vi "JY .vi"() -> ()   [LabVIEW 2018]
doc: "This VI is an example on how to use the HORIBA Jobin Yvon Monochromator control VIs. To use this VI, press the Run button in LabVIEW.\n\nThe VI will retreive all configured monochromators from the computer's resgistry.\n\nSelect the desired monochromator from the Mono ID combo box and press the Connect button to start communications with that device. If the Force Initialization button is enabled, the monochromator will start its automatic calibration routine. If the Force Initialization button is not enabled, the sofwtare will keep the monochromator in its current positions.\n\nAfter connecting to the instrumnet, the VI will retreive the current positions of all movable motors in the system. This will continue until the Move To Target Position or Stop buttons are pressed.\n\nMove to Target Positions will move the monochromator to the postions entered in the indicators of the VI.\n\nStop will stop running the VI."
uses:
  <vilib>/Utility/file.llb/Write Delimited Spreadsheet (DBL).vi
panel:
  out "最终存储路径":path
  in  "Commande tab":enum32{"Settings", "Trigger In", "Infos"}(tab)
  in  "Integration time (ms) :":i16=10
  in  "Number of Areas :":u16=1 min=1 step=1
  in  "ADC":u16(ring) caption="Device Name" items=["20 kHz       ", " 1 MHz       ", " 1 MHz Ultra "]
  in  "GAIN":u16(ring) caption="Device Name" items=["High Light", "Best Dynamic Range", "High Sensitivity"]
  in  "Device Name":u16(ring) items=["Synapse CCD (Lateral)", "Synapse_IGA (Axial)"]
  out "Uniques ID":u16(ring) items=["CCD1", "CCD2"]
  in  "Reformat":bool
  in  "Signal type :":enum16{"TTL Rising Edge", "TTL Falling Edge"}(ring)=enum."TTL Falling Edge"
  in  "Trigger Type :":enum16{"On Start", "Per Acquisition"}(ring)
  in  "Enable InputTriggers :":bool
  out "DataSize":i32=262144
  out "Y Pixels:":i32=256
  out "X Pixels:":i32=1024
  out "Firmware\nVersion":string="V1.20 CCD_4000"
  out "Intensity Graph":dbl[][](graph)
  out "initialized ccd":bool
  in  "Continuous":bool
  in  "CCD Busy":bool
  out "indicator":string
  in  "Close":bool=TRUE
  in  "Setup":bool
  in  "Temperature":bool
  in  "Acquire":bool
  in  "Shutter Enable":bool=TRUE
  out "Acq Time(ms)":u32=2010
  in  "initialize":bool
  in  "Target\nFront Entrance":dbl
  in  "Exit Mirror":u16(ring)=3 caption="Target Position Exit Mirror" items=["Front"=2, "Side"=3]
  in  "Entrance Mirror":u16(ring)=2 caption="Target Position\nEntrance Mirror" items=["Front"=2, "Side"=3]
  in  "Target Grating":string(combo)="2"
  in  "Target WL":dbl=898.0
  in  "Move To\nTarget Positions":bool
  out "Units":string="nm"
  in  "Connect":bool
  out "Initialized JY":bool=TRUE
  out "Current UniqueID":string="Mono4"
  in  "Force\nInitialization":bool=TRUE
  out "Units":string="mm"
  out "Front Entrance":dbl
  out "Exit Mirror\nPosition":i32(ring)=2 items=["EntranceMirror", "ExitMirror", "Front", "Side"]
  out "Entrance Mirror\nPosition":i32(ring)=2 items=["EntranceMirror", "ExitMirror", "Front", "Side"]
  out "Current Description":string="1" caption="Description"
  out "Grating Index":i32=1
  out "Current Grating":dbl=1200.0
  out "Current WL":dbl=897.9988
  in  "Mono ID":string(combo)="Mono1"
  in  "trigEventString":string
  in  "trigSigTypeString":string
  in  "trigAddress":i32
  out "ADC Number":i32[](array[numeric])=[0, 1, 2, 3, 4]
  out "Gain Number":i32[](array[numeric])=[10, 11, 12, 13, 8, 2]
  out "temp graph":dbl(graph)=66.11766439999997
  out "areas :":i32[][](array[numeric])=[[1], [1], [1], [1024], [256], [1], [1]]
  out "Gratings":dbl[](array[numeric])=[1200.0, 300.0]
  out "error out":errorcluster
  # "JY Control"
  # "Setup"
  # "Grating / Wavelength Control"
  # "Slits"
  # "Swing Mirrors"
  # "CCD Control"
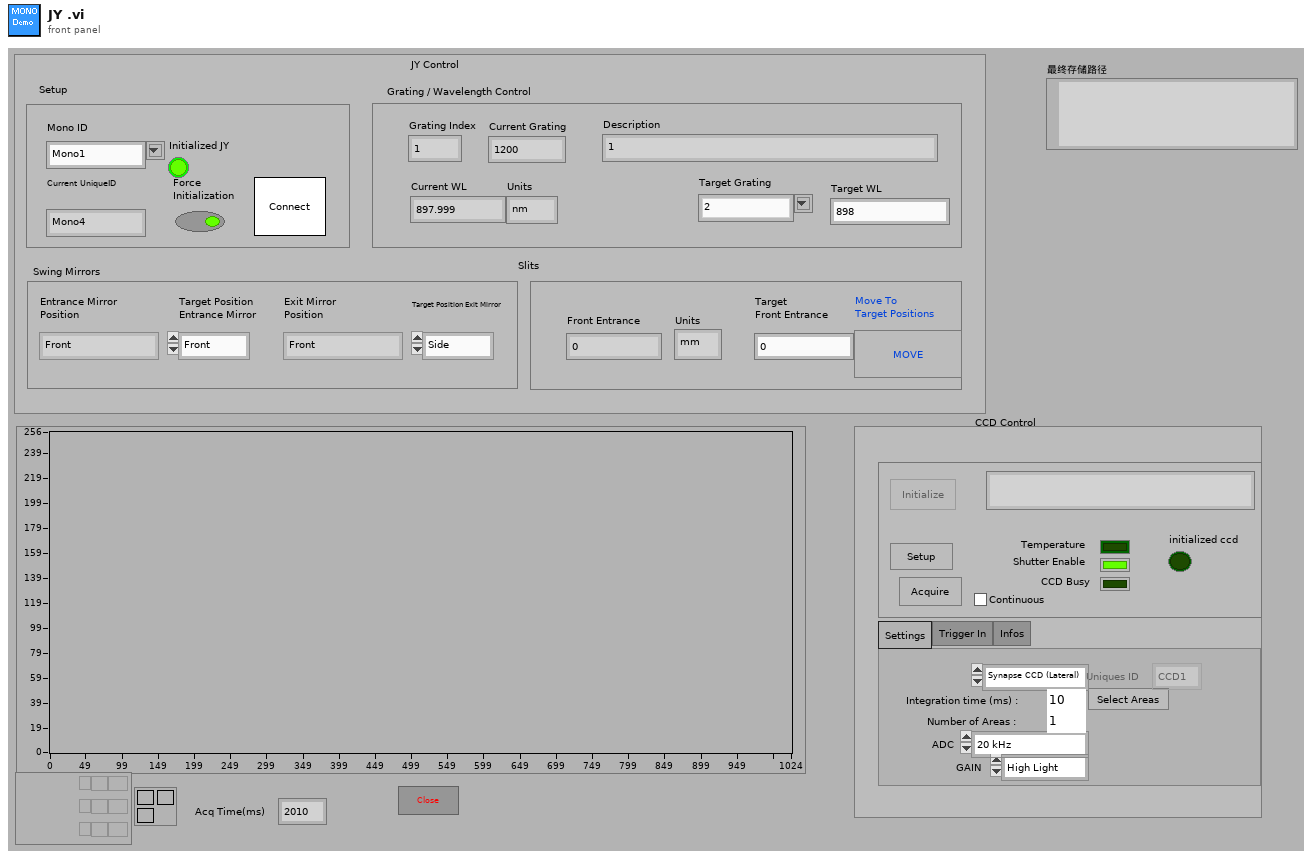
[diagram p1: front panel]
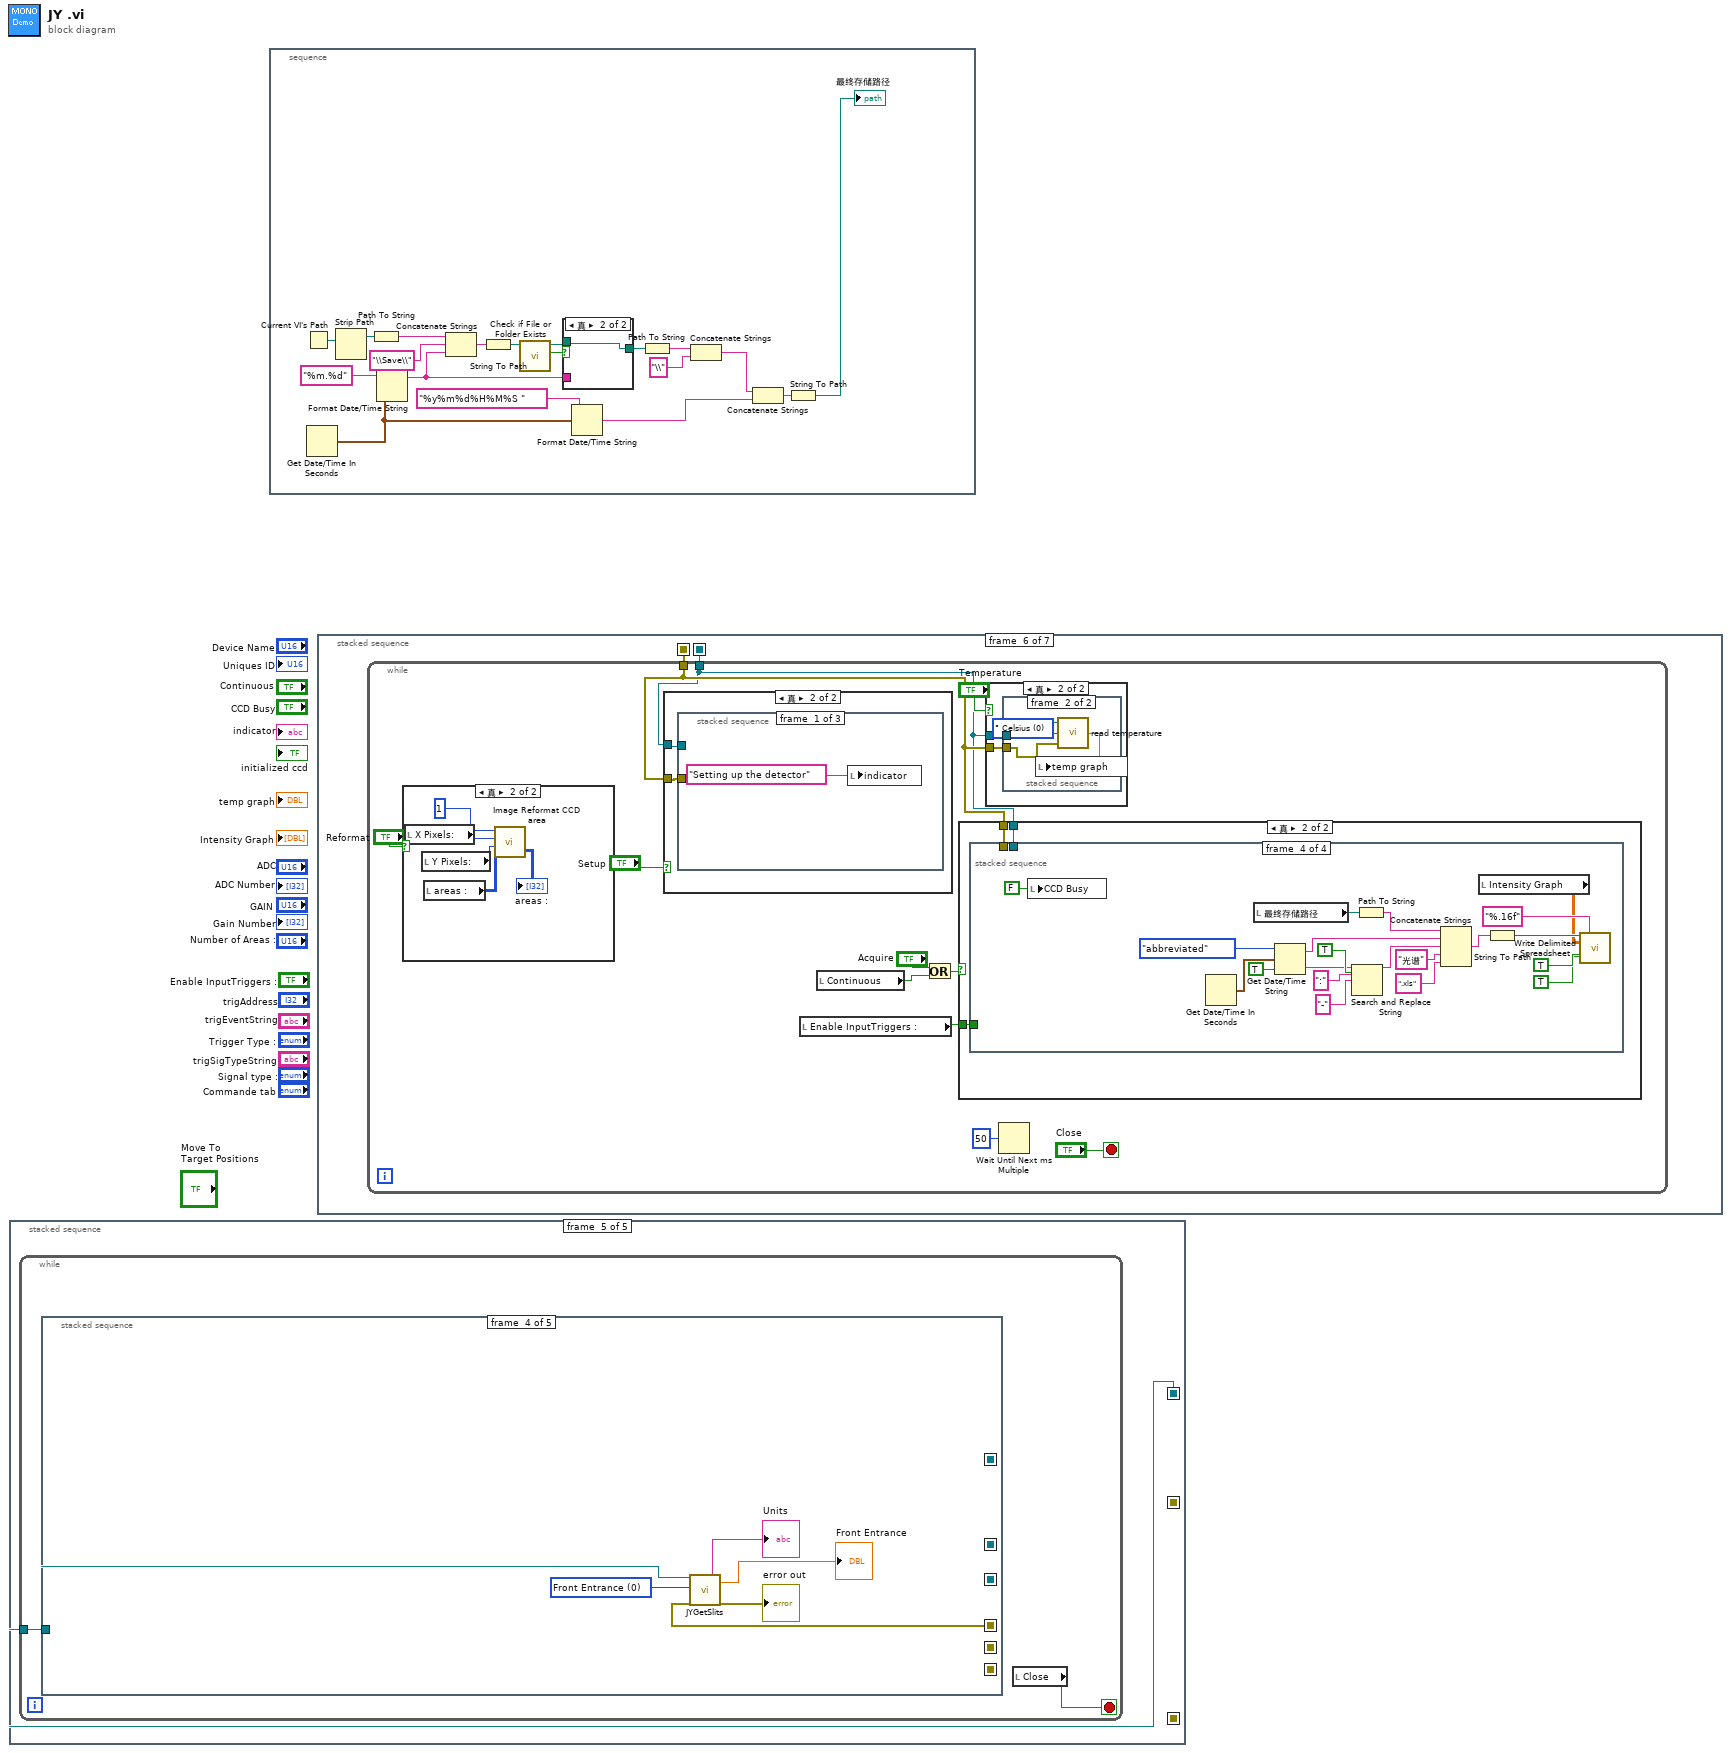
[diagram p0: block diagram]
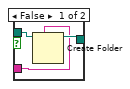
[diagram p2: hidden frame]
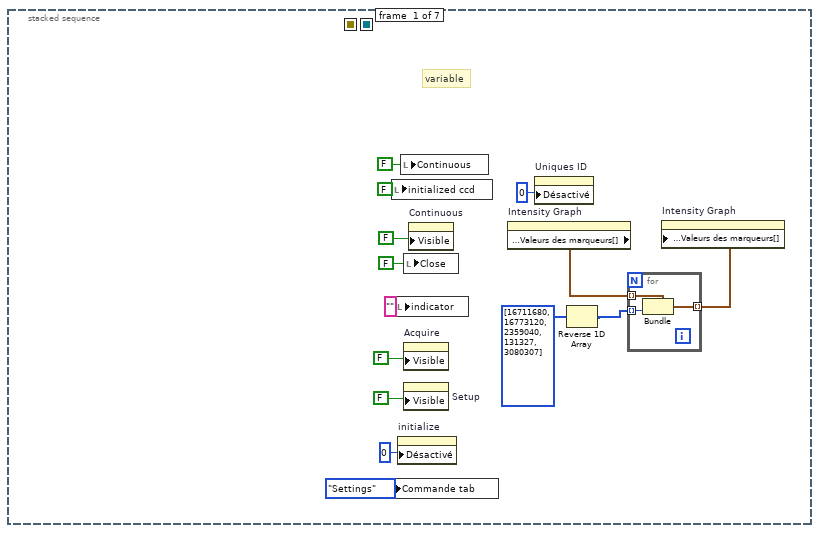
[diagram p3: hidden frame]
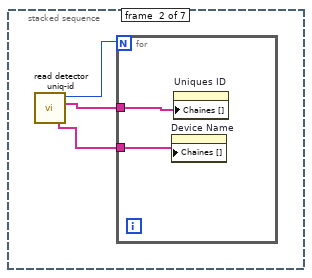
[diagram p4: hidden frame]
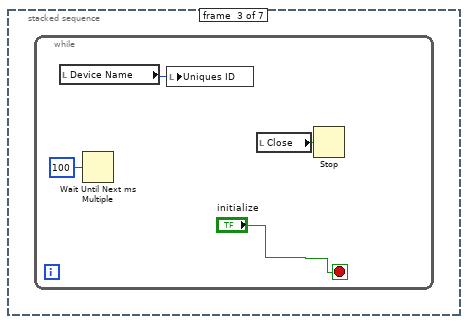
[diagram p5: hidden frame]
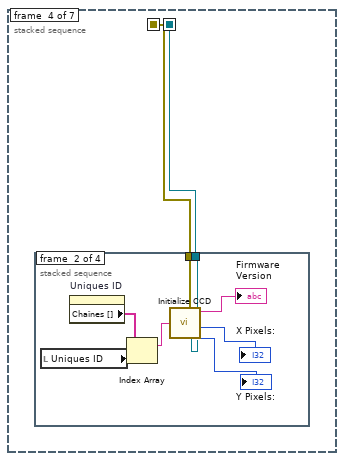
[diagram p6: hidden frame]
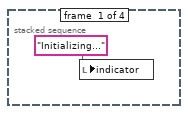
[diagram p7: hidden frame]
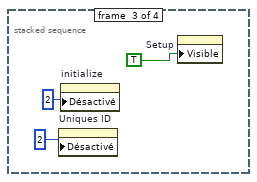
[diagram p8: hidden frame]
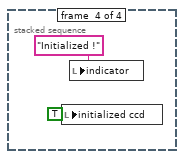
[diagram p9: hidden frame]
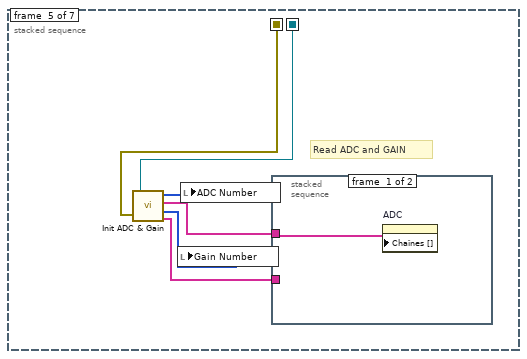
[diagram p10: hidden frame]
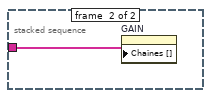
[diagram p11: hidden frame]
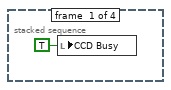
[diagram p13: hidden frame]
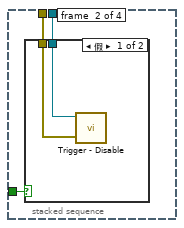
[diagram p14: hidden frame]
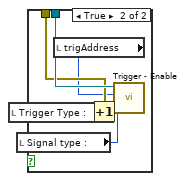
[diagram p15: hidden frame]
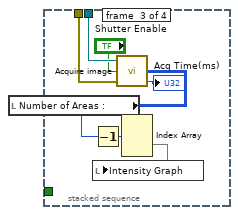
[diagram p16: hidden frame]
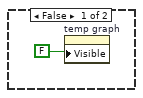
[diagram p17: hidden frame]
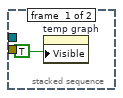
[diagram p18: hidden frame]
diagram:
  n1 = stacked-sequence {
    seq-local: [_ _ w10 _ _] -> [_ _ _ w20 w25]
    seq-local: [_ _ w9 _ _] -> [_ _ _ w19 _]
    seq-local: [_ _ _ w18 _] -> [_ _ _ _ _]
    frame #0 {
      n2 = call "Get Monos From Config Browser.vi"() -> ("UniqueIDs"=w5:string[], "Mono ID"=w6:string[])  [unwired: 3 in, 1 out]
      n3 = Build Cluster Array(w6, w5) -> (w3:cluster{"String":string, "String":string}[])
      n4 = property on="Mono ID" class="CmbBox"("Strings And Values []"=w3) -> ()  [unwired: 2 in, 2 out]
      n5 = Index Array(array=w3, index=0) -> (element=w4:cluster{"String":string, "String":string})
      n6 = Unbundle(w4) -> ("String"=w1:string)  [unwired: 1 out]
      "Current UniqueID" <- w1
      n7 = local write "Mono ID"(w1) -> ()
    }
    frame #1 {
      n8 = while {
        stop <- "Connect" stop-if-true
        n9 = local read "Mono ID"() -> (w7:string)
        n10 = local write "Current UniqueID"(w7) -> ()
      }
    }
    frame #2 {
      n11 = local read "Mono ID"() -> (w12:string)
      n12 = call "JYInitMono.vi"("Unique ID"=w12, "Force Init"="Force\nInitialization") -> ("Refnum out"=w10:refnum<k7>, "Initialized"=→"Initialized JY":bool, "error out"=w9:errorcluster)  [unwired: 9 in, 2 out]
    }
    frame #3 {
      n13 = call "Show Current Grating.vi"("Refnum in"=w20, "error in (no error)"=w19) -> ("Gratings"=w21:dbl[], "Grating Index"=w15:i32, "Current Grating"=w17:dbl, "Current Description"=w14:string, "error out"=w18:errorcluster)  [unwired: 5 in, 4 out]
      "Gratings" <- w21
      n14 = local write "Current Grating"(w17) -> ()
      n15 = local write "Current Description"(w14) -> ()
      n16 = Number To Decimal String(number=w21) -> (decimal integer string=w23:string[])  [unwired: 1 in]
      n17 = Number To Decimal String(number=w15) -> (decimal integer string=w16:string)  [unwired: 1 in]
      n18 = property on="Target Grating" class="CmbBox"("Value"=w16) -> ()  [unwired: 2 in, 2 out]
      n19 = Build Cluster Array(w23, string[] ["1", "2", "3"]) -> (w24:cluster{"Numeric":string, string}[])
      n20 = property on="Target Grating" class="CmbBox"("Strings And Values []"=w24) -> ()  [unwired: 2 in, 2 out]
    }
    frame #4 {
      n21 = while {
        tunnel: w25 -> [w27]
        stop <- w26 stop-if-true
        n22 = stacked-sequence {
          seq-local: [w31 _ _ _ _] -> [_ w38 w49 _ w56]
          seq-local: [w30 _ _ _ _] -> [_ w37 w48 _ _]
          seq-local: [_ w36 _ _ _] -> [_ _ _ _ _]
          seq-local: [_ w35 _ _ _] -> [_ _ _ _ _]
          seq-local: [_ _ w41 _ _] -> [_ _ _ _ _]
          seq-local: [_ _ w40 _ _] -> [_ _ _ w51 _]
          tunnel: w27 -> [w29 _ _ w52 _]
          frame #0 {
            n23 = call "Show Current Grating.vi"("Refnum in"=w29) -> ("Grating Index"=→"Grating Index":i32, "Current Grating"=→"Current Grating":dbl, "Current Description"=→"Current Description":string, "error out"=w30:errorcluster, "JYMONOLib.IJYMonoReqd"=w31:refnum<k7>)  [unwired: 6 in, 4 out]
          }
          frame #1 {
            n24 = call "JYGetCurrentWL.vi"("error in (no error)"=w37, "JYMONOLib.IJYMonoReqd"=w38) -> ("error out"=w35:errorcluster, "Units"=→"Units":string, "Current WL"=→"Current WL":dbl, "JYMONOLib.IJYMonoReqd 2"=w36:refnum<k7>)  [unwired: 6 in]
          }
          frame #2 {
            w46 = u16 1 items=["Entrance", "Exit"] ("Mirror Number")
            w47 = u16 0 items=["Entrance", "Exit"] ("Mirror Number")
            n25 = call "JYGetMirrorPos.vi"("error in (no error)"=w48, "Mirror"=w47, "Refnum In"=w49) -> ("error out"=w44:errorcluster, "Current Mirror Position"=→"Entrance Mirror\nPosition":i32, "Refnum Out"=w45:refnum<k7>)  [unwired: 1 in]
            n26 = call "JYGetMirrorPos.vi"("error in (no error)"=w44, "Mirror"=w46, "Refnum In"=w45) -> ("error out"=w40:errorcluster, "Current Mirror Position"=→"Exit Mirror\nPosition":i32, "Refnum Out"=w41:refnum<k7>)  [unwired: 1 in]
          }
          frame #3 {
            w54 = u16 0 items=["Front Entrance", "Side Entrance", "Front Exit", "Side Exit", "First Intermediate", "Second Intermediate"] ("Slit")
            n27 = call "JYGetSlits.vi"("MonoRefNum IN"=w52, "Slit"=w54, "error in (no error)"=w51) -> ("Units"=→"Units":string, "Slit Width"=→"Front Entrance":dbl, "error out"=→"error out":errorcluster)  [unwired: 13 in, 1 out]
          }
          frame #4 {
            n28 = local read "Move To\nTarget Positions"() -> (w57:bool)
            n29 = case shown="真" w57 {
              tunnel: w56 -> [_ w58]
              frame False {
              }
              frame True {
                n30 = stacked-sequence {
                  seq-local: [w60 _ _ _] -> [_ w66 _ _]
                  seq-local: [_ w64 _ _] -> [_ _ w81 _]
                  seq-local: [_ _ w68 _] -> [_ _ _ w87]
                  seq-local: [_ _ _ w84] -> [_ _ _ _]
                  tunnel: w58 -> [w62 w65 w79 w88]
                  frame #0 {
                    n31 = property on="Target Grating" class="CmbBox"() -> ("Value"=w59:string)  [unwired: 2 in, 2 out]
                    n32 = local read "error out"() -> (w61:errorcluster)
                    n33 = Decimal String To Number(string=w59) -> (number=w63:i32)  [unwired: 2 in, 1 out]
                    n34 = call "JYTurret.vi"("error in (no error)"=w61, "Grating Index"=w63, "JYMONOLib.IJYMonoReqd"=w62) -> ("error out"=w60:errorcluster)  [unwired: 2 out]
                  }
                  frame #1 {
                    # "Move Grating to Target Position"
                    n35 = call "JYMoveToWavelength.vi"("error in (no error)"=w66, "Target WL"="Target WL", "RefNum In"=w65) -> ("error out"=w64:errorcluster)  [unwired: 1 in, 2 out]
                  }
                  frame #2 {
                    w74 = u16 1 items=["Entrance", "Exit"] ("Mirror Number")
                    w73 = u16 0 items=["Entrance", "Exit"] ("Mirror Number")
                    w80 = u16 1 items=["Entrance", "Exit", "Front", "Side"] ("Mirror Number")
                    w83 = u16 0 items=["Entrance", "Exit", "Front", "Side"] ("Mirror Number")
                    # "Move Mirrors"
                    n36 = call "JYMirrorMove.vi"("error in (no error)"=w81, "Mirror Position"="Entrance Mirror", "Mirror Number"=w83, "RefNum In"=w79) -> ("error out"=w78:errorcluster)  [unwired: 6 in, 1 out]
                    n37 = call "JYMirrorMove.vi"("error in (no error)"=w78, "Mirror Position"="Exit Mirror", "Mirror Number"=w80, "RefNum In"=w79) -> ("error out"=w71:errorcluster, "MonoRefNum Out"=w72:refnum<k7>)  [unwired: 6 in]
                    n38 = call "JYGetMirrorPos.vi"("error in (no error)"=w71, "Mirror"=w73, "Refnum In"=w72) -> ("error out"=w76:errorcluster, "Current Mirror Position"=w70:i32, "Refnum Out"=w75:refnum<k7>)  [unwired: 1 in]
                    n39 = local write "Entrance Mirror\nPosition"(w70) -> ()
                    n40 = call "JYGetMirrorPos.vi"("error in (no error)"=w76, "Mirror"=w74, "Refnum In"=w75) -> ("error out"=w68:errorcluster, "Current Mirror Position"=w69:i32)  [unwired: 1 in, 1 out]
                    n41 = local write "Exit Mirror\nPosition"(w69) -> ()
                  }
                  frame #3 {
                    w86 = u16 0 items=["Front Entrance", "Side Entrance", "Front Exit", "Side Exit", "First Intermediate", "Second Intermediate"] ("Slit")
                    # "Set New Slit Positions"
                    n42 = call "JYSlits.vi"("JYMONOLib.IJYMonoReqd"=w88, "Slit"=w86, "error in (no error)"=w87, "Slit Width"="Target\nFront Entrance") -> ("error out"=w84:errorcluster)  [unwired: 1 in, 1 out]
                  }
                }
              }
            }
          }
        }
        n43 = local read "Close"() -> (w26:bool)
      }
    }
  }
  n44 = stacked-sequence {
    frame #0 {
      n45 = Current VI's Path() -> (path=w105:path)
      n46 = Get Date/Time In Seconds() -> (seconds since 1Jan1904=w102:timestamp)
      n47 = Strip Path(path=w105) -> (stripped path=w104:path)  [unwired: 1 out]
      n48 = Path To String(path=w104) -> (string=w101:string)
      n49 = Format Date/Time String(time format string (%c)="%m.%d" ("时间格式字符串(%c)"), seconds (now)=w102) -> (date/time string=w94:string)  [unwired: 1 in]
      n50 = Concatenate Strings(w101, "\\Save\\" ("字符串"), w94) -> (w99:string)
      n51 = String To Path(string=w99) -> (path=w98:path)
      n52 = call <vilib>:"Check if File or Folder Exists.vi"("path"=w98) -> ("file or folder exists?"=w97:bool, "dup path"=w95:path)  [unwired: 8 in, 1 out]
      n53 = case shown="真" w97 {
        tunnel: [w110 w111] -> w96
        tunnel: w95 -> [w109 w111]
        tunnel: w94 -> [w108 _]
        frame False {
          n54 = Create Folder(prompt (Create Folder)=w108, path (use dialog)=w109) -> (created path=w110:path)  [unwired: 1 in, 2 out]
        }
        frame True {
        }
      }
      n55 = Format Date/Time String(time format string (%c)="%y%m%d%H%M%S " ("时间格式字符串(%c)"), seconds (now)=w102) -> (date/time string=w90:string)  [unwired: 1 in]
      n56 = Path To String(path=w96) -> (string=w93:string)
      n57 = Concatenate Strings(w93, "\\" ("字符串")) -> (w91:string)
      n58 = Concatenate Strings(w91, w90) -> (w107:string)
      n59 = String To Path(string=w107) -> (path=→"最终存储路径":path)
    }
  }
  n60 = stacked-sequence {
    seq-local: [_ _ _ w139 _ _ _] -> [_ _ _ _ w155 w163 w249]
    seq-local: [_ _ _ w138 _ _ _] -> [_ _ _ _ w154 w162 w250]
    frame #0 {
      # "variable"
      n61 = local write "Commande tab"(enum32{"Settings", "Trigger In", "Infos"}."Settings" ("Commande tab")) -> ()
      n62 = local write "initialized ccd"(FALSE ("initialized ?")) -> ()
      n63 = local write "indicator"("" ("indicator")) -> ()
      n64 = property on="initialize" class="Bool"("Désactivé"=u8 0) -> ()  [unwired: 2 in, 2 out]
      n65 = local write "Continuous"(FALSE ("Continuous")) -> ()
      n66 = local write "Close"(FALSE ("Close")) -> ()
      n67 = property on="Acquire" class="Bool"("Visible"=FALSE) -> ()  [unwired: 2 in, 2 out]
      n68 = property on="Setup" class="Bool"("Visible"=FALSE) -> ()  [unwired: 2 in, 2 out]
      n69 = property on="Continuous" class="Bool (严格)"("Visible"=FALSE) -> ()  [unwired: 2 in, 2 out]
      n70 = property on="Intensity Graph" class="IntGraph (严格)"() -> ("Échelle des Z.Valeurs des marqueurs[]"=w115:cluster{dbl, u32}[])  [unwired: 2 in, 2 out]
      n71 = property on="Uniques ID" class="Ring (严格)"("Désactivé"=u8 0) -> ()  [unwired: 2 in, 2 out]
      n72 = Reverse 1D Array(array=u32[] [16711680, 16773120, 2359040, 131327, 3080307] ("Sous-tableau")) -> (reversed array=w116:u32[])
      n73 = for {
        tunnel: w116 -> [w128] mode=indexing
        tunnel: [w127] -> w114 mode=indexing
        tunnel: w115 -> [w126] mode=indexing
        n74 = Bundle(cluster=w126, w128) -> (w127:cluster{dbl, u32})  [unwired: 1 out]
      }
      n75 = property on="Intensity Graph" class="IntGraph (严格)"("Échelle des Z.Valeurs des marqueurs[]"=w114) -> ()  [unwired: 2 in, 2 out]
    }
    frame #1 {
      n76 = call <userlib>:"read detector uniq-id.vi"() -> ("nbr of components"=w131:i32, "UniqueID"=w130:string[], "Name"=w129:string[])  [unwired: 4 out]
      n77 = for {
        N: w131 -> [_]
        tunnel: w130 -> [w133]
        tunnel: w129 -> [w132]
        n78 = property on="Device Name" class="Ring (严格)"("Chaînes []"=w132) -> ()  [unwired: 2 in, 2 out]
        n79 = property on="Uniques ID" class="Ring (严格)"("Chaînes []"=w133) -> ()  [unwired: 2 in, 2 out]
      }
    }
    frame #2 {
      n80 = while {
        stop <- "initialize" stop-if-true
        n81 = local read "Device Name"() -> (w136:u16)
        n82 = Wait Until Next ms Multiple(millisecond multiple=u32 100 ("n millisecondes")) -> ()  [unwired: 1 out]
        n83 = local write "Uniques ID"(w136) -> ()
        n84 = local read "Close"() -> (w134:bool)
        n85 = Stop(stop? (T)=w134) -> ()
      }
    }
    frame #3 {
      n86 = stacked-sequence {
        tunnel: [_ w145 _ _] -> w139
        tunnel: [_ w144 _ _] -> w138
        frame #0 {
          n87 = local write "indicator"("Initializing..." ("indicator")) -> ()
        }
        frame #1 {
          n88 = local read "Uniques ID"() -> (w142:u16)
          n89 = property on="Uniques ID" class="Ring (严格)"() -> ("Chaînes []"=w143:string[])  [unwired: 2 in, 2 out]
          n90 = Index Array(array=w143, index=w142) -> (element=w141:string)
          n91 = call <userlib>:"Initialize CCD.vi"("Unique id:"=w141) -> ("activeYPixels"=→"Y Pixels:":i32, "JYCCDLib.IJYCCDReqd"=w144:refnum<k7>, "activeXPixels"=→"X Pixels:":i32, "sortie d'erreur"=w145:errorcluster, "FirmwareVersion"=→"Firmware\nVersion":string)  [unwired: 3 out]
        }
        frame #2 {
          n92 = property on="Uniques ID" class="Ring (严格)"("Désactivé"=u8 2) -> ()  [unwired: 2 in, 2 out]
          n93 = property on="initialize" class="Bool"("Désactivé"=u8 2) -> ()  [unwired: 2 in, 2 out]
          n94 = property on="Setup" class="Bool"("Visible"=TRUE) -> ()  [unwired: 2 in, 2 out]
        }
        frame #3 {
          n95 = local write "initialized ccd"(TRUE ("initialized ?")) -> ()
          n96 = local write "indicator"("Initialized !" ("indicator")) -> ()
        }
      }
    }
    frame #4 {
      # "Read ADC and GAIN"
      n97 = call <userlib>:"Init ADC & Gain.vi"("JYCCDLib.IJYCCDReqd"=w154, "input error"=w155) -> ("ADC Number"=w157:i32[], "ADC description"=w159:string[], "Gain Number"=w156:i32[], "Gain description"=w158:string[])
      n98 = local write "Gain Number"(w156) -> ()
      n99 = local write "ADC Number"(w157) -> ()
      n100 = stacked-sequence {
        tunnel: w159 -> [w160 _]
        tunnel: w158 -> [_ w161]
        frame #0 {
          n101 = property on="ADC" class="Ring (严格)"("Chaînes []"=w160) -> ()  [unwired: 2 in, 2 out]
        }
        frame #1 {
          n102 = property on="GAIN" class="Ring (严格)"("Chaînes []"=w161) -> ()  [unwired: 2 in, 2 out]
        }
      }
    }
    frame #5 {
      n103 = while {
        tunnel: w162 -> [w165]
        tunnel: w163 -> [w166]
        stop <- "Close" stop-if-true
        n104 = case shown="真" "Reformat" {
          frame False {
          }
          frame True {
            n105 = local read "X Pixels:"() -> (w228:i32)
            n106 = local read "Y Pixels:"() -> (w230:i32)
            n107 = local read "areas :"() -> (w226:i32[][])
            n108 = call "Image Reformat CCD area.vi"("areas :"=w226, "Y Pixels:"=w230, "X Pixels:"=w228, "numAreas"=1) -> ("areas"=→"areas :":i32[][])  [unwired: 1 out]
          }
        }
        n109 = case shown="真" "Setup" {
          tunnel: w166 -> [_ w231]
          tunnel: w165 -> [_ w232]
          frame False {
          }
          frame True {
            n110 = stacked-sequence {
              tunnel: w231 -> [_ w246 _]
              tunnel: w232 -> [_ w243 _]
              frame #0 {
                n111 = local write "indicator"("Setting up the detector" ("indicator")) -> ()
              }
              frame #1 {
                w244 = 1 items=["JYMCD_ACQ_FORMAT_IMAGE", "JYMCD_ACQ_FORMAT_SCAN"] ("Acquisition type")
                n112 = local read "Gain Number"() -> (w238:i32[])
                n113 = local read "GAIN"() -> (w234:u16)
                n114 = local read "ADC Number"() -> (w239:i32[])
                n115 = local read "ADC"() -> (w235:u16)
                n116 = Index Array(array=w238, index=w234) -> (element=w236:i32)
                n117 = Index Array(array=w239, index=w235) -> (element=w237:i32)
                n118 = local read "Number of Areas :"() -> (w241:u16)
                n119 = local read "areas :"() -> (w242:i32[][])
                n120 = call <userlib>:"Setup CCD.vi"("numAreas"=w241, "areas :"=w242, "JYCCDLib.IJYCCDReqd"=w243, "entrée d'erreur (pas d'erreur)"=w246, "Acquisition type"=w244, "Gain"=w236, "Select ADC"=w237, "Integration time(ms)"="Integration time (ms) :") -> ("DataSize"=→"DataSize":i32)  [unwired: 1 out]
              }
              frame #2 {
                w247 = TRUE ("Visible")
                n121 = property on="Acquire" class="Bool"("Visible"=w247) -> ()  [unwired: 2 in, 2 out]
                n122 = local write "indicator"("Ready !" ("indicator")) -> ()
                n123 = property on="Continuous" class="Bool (严格)"("Visible"=w247) -> ()  [unwired: 2 in, 2 out]
              }
            }
          }
        }
        n124 = local read "Enable InputTriggers :"() -> (w164:bool)
        n125 = local read "Continuous"() -> (w167:bool)
        n126 = Or(x="Acquire", y=w167) -> (x .or. y?=w169:bool)
        n127 = case shown="真" w169 {
          tunnel: w165 -> [_ w177]
          tunnel: w166 -> [_ w176]
          tunnel: w164 -> [_ w175]
          frame False {
          }
          frame True {
            n128 = stacked-sequence {
              tunnel: w177 -> [_ w180 w197 _]
              tunnel: w176 -> [_ w179 w196 _]
              tunnel: w175 -> [_ w181 _ _]
              frame #0 {
                n129 = local write "CCD Busy"(TRUE ("CCD Busy")) -> ()
              }
              frame #1 {
                n130 = case shown="假" w181 {
                  tunnel: w180 -> [w183 w189]
                  tunnel: w179 -> [w182 w188]
                  frame False {
                    n131 = call <userlib>:"Trigger - Disable.vi"("Error In"=w182, "JYCCDLib.IJYCCDReqd"=w183) -> ()  [unwired: 6 out]
                  }
                  frame True {
                    n132 = local read "Trigger Type :"() -> (w186:enum16{"On Start", "Per Acquisition"})
                    n133 = local read "Signal type :"() -> (w185:enum16{"TTL Rising Edge", "TTL Falling Edge"})
                    n134 = local read "trigAddress"() -> (w187:i32)
                    n135 = Increment(x=w186) -> (x+1=w184:enum16{"On Start", "Per Acquisition"})
                    n136 = call <userlib>:"Trigger - Enable.vi"("Error In"=w188, "sigType"=w185, "event"=w184, "trigAddress"=w187, "JYCCDLib.IJYCCDReqd"=w189) -> ()  [unwired: 3 out]
                  }
                }
              }
              frame #2 {
                n137 = local read "Number of Areas :"() -> (w191:u16)
                n138 = Decrement(x=w191) -> (x-1=w193:u16)
                n139 = call "Acquire image.vi"("error in"=w196, "ShutterOpen"="Shutter Enable", "JYCCDLib.IJYCCDReqd"=w197) -> ("Acq Time(ms)"=→"Acq Time(ms)":u32, "Datas"=w194:i32[][][])  [unwired: 1 out]
                n140 = Index Array(array=w194, index (dim 0)=w193) -> (element=w192:i32[][])  [unwired: 2 in]
                n141 = local write "Intensity Graph"(w192) -> ()
              }
              frame #3 {
                n142 = local write "CCD Busy"(FALSE ("CCD Busy")) -> ()
                n143 = Get Date/Time In Seconds() -> (seconds since 1Jan1904=w206:timestamp)
                n144 = local read "最终存储路径"() -> (w215:path)
                n145 = Get Date/Time String(date format (0)=enum16{"short", "long", "abbreviated"}."abbreviated" ("日期格式(0)"), seconds (now)=w206, want seconds? (F)=TRUE ("需要秒？(F)")) -> (date string=w214:string, time string=w209:string)
                n146 = Search and Replace String(replace all?=TRUE ("替换全部？(F)"), input string=w209, search string=":" ("搜索字符串"), replace string="-" ("替换字符串(\"\")")) -> (result string=w213:string)  [unwired: 4 in, 3 out]
                n147 = Path To String(path=w215) -> (string=w216:string)
                n148 = Concatenate Strings(w216, w214, w213, "光谱" ("字符串"), ".xls" ("字符串")) -> (w199:string)
                n149 = local read "Intensity Graph"() -> (w198:dbl[][])
                n150 = String To Path(string=w199) -> (path=w203:path)
                n151 = call-poly <vilib>:"Write Delimited Spreadsheet.vi"("file path (dialog if empty)"=w203, "format (%.3f)"="%.16f", "2D data"=w198, "append to file? (new file:F)"=TRUE ("append to file? (F)"), "transpose? (no:F)"=TRUE ("transpose? (F)")) -> ()  [unwired: 9 in, 2 out]
              }
            }
          }
        }
        n152 = case shown="真" "Temperature" {
          tunnel: w165 -> [_ w220]
          tunnel: w166 -> [_ w219]
          frame False {
            n153 = property on="temp graph" class="WFChart (严格)"("Visible"=FALSE) -> ()  [unwired: 2 in, 2 out]
          }
          frame True {
            n154 = stacked-sequence {
              tunnel: w220 -> [_ w225]
              tunnel: w219 -> [_ w224]
              frame #0 {
                n155 = property on="temp graph" class="WFChart (严格)"("Visible"=TRUE) -> ()  [unwired: 2 in, 2 out]
              }
              frame #1 {
                w223 = u16 0 items=["° Celsius", "Kelvin", "° Farenheit"] ("units")
                n156 = call <userlib>:"read temperature.vi"("entrée d'erreur (pas d'erreur)"=w224, "units"=w223, "JYCCDLib.IJYCCDReqd"=w225) -> ("Current Temperature"=w222:dbl)
                n157 = local write "temp graph"(w222) -> ()
              }
            }
          }
        }
        n158 = Wait Until Next ms Multiple(millisecond multiple=u32 50 ("n millisecondes")) -> ()  [unwired: 1 out]
      }
    }
    frame #6 {
      n159 = Close Reference(reference=w250, error in (no error)=w249) -> ()  [unwired: 1 out]
    }
  }
